vi "Own20261012_SetLoopTunnelConditional.vi"() -> ()   [LabVIEW 2024]
panel:
  out "error out":errorcluster caption="错误输出"
  in  "is_conditional":bool
  in  "tunnel_id":u32
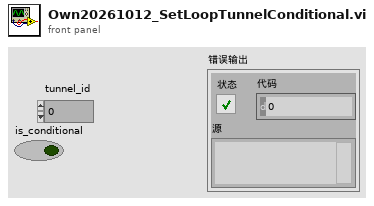
[diagram p1: front panel]
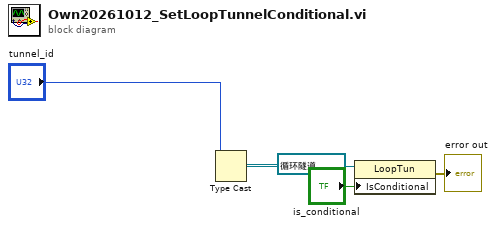
[diagram p0: block diagram]
diagram:
  n1 = Type Cast(type=refnum<vi> refnum ("引用"), x="tunnel_id") -> (*(type *) &x=w3:refnum<vi>)
  n2 = property class="LoopTun"(reference=w3, "IsConditional"="is_conditional") -> (error out=→"error out":errorcluster)  [unwired: 1 in, 1 out]
